vi "PicoScope5000aExampleStreamingMSO.vi"() -> ()   [LabVIEW 2010]
doc: "This example demonstrates how to use the PicoScope Labview library to stream data from a PicoScope 5000 Series Device"
uses:
  <vilib>/Waveform/DWDTOps.llb/DWDT Analog to Digital.vi
  PicoScope5000aLib/PicoScope5000aAnalogChannelSettings.ctl
  PicoScope5000aLib/PicoScope5000aDigitalChannelSettings.ctl
panel:
  in  "Port 0 Settings":T1={"Enabled"=FALSE, "Logic Level"=9830} {"Logic Level" items=["1.5V TTL"=9830, "2.5V CMOS"=16383]}
  in  "Channel A Settings":T2={"Enabled"=TRUE, "Coupling"=1, "Range"=6, "Analogue Offset"=0.0, "Bandwidth Limit"=0} {"Bandwidth Limit" items=["Full", "20MHz"]; "Range" items=["10 mV", "20 mV", "50 mV", "100 mV", "200 mV", "500 mV", "1 V", "2 V", "5 V", "10 V", "20 V"]; "Coupling" items=["AC", "DC"]}
  in  "Write ChA to file":bool
  out "Analog Channels":T3(graph)={0, "DownSample Interval (sec)"=1.600000020814234e-08, "Data"=[]}
  out "Raw Sample Interval (sec)":dbl format="%#.5p"
  out "Max ADC value":i16=32512
  out "Chunk time (ms)":u32
  out "Elapsed time (sec)":dbl
  in  "Data file":path=path "PicoScope5000aExampleStreaming ChA Data"
  out "Queue depth":i32(graph)=3
  out "queue depth":i32
  in  "Buffer and Transfer Settings":T4={"startIndex"=0, "Samples"=1000000, "Down Sample Ratio"=1, "Down-Sample Mode"=0} {"Down-Sample Mode" items=["None"=0, "Aggregate"=1, "Decimate"=2, "Average"=4]; "Down Sample Ratio" step=1; "Samples" format="%_6p"}
  out "USB Powered":bool=TRUE
  out "USB 3.0 device on non-USB 3.0 Port":bool
  out "TriggeredAt (In Buffer)":u32 format="%#.6p"
  out "TriggeredAt (Total samples)":u32 format="%#.6p"
  in  "Acquisition Settings":T5={"Auto Stop"=TRUE, "Desired Sample Interval"=1, "Pre-trigger Samples"=0, "Post-trigger Samples"=1000000, "Down-Sample Ratio"=1, "Down-Sample Mode"=0, "Time Units"=3} {"Time Units" items=["Nanoseconds (ns)"=2, "Microseconds (us)"=3, "Milliseconds (ms)"=4, "Seconds (s)"=5]; "Down-Sample Mode" items=["None"=0, "Aggregate"=1, "Decimate"=2, "Average"=4]; "Post-trigger Samples" format="%#.6p"; "Pre-trigger Samples" format="%#_6p"}
  out "Port 0":digitalwaveform(graph)={"t0"=timestamp(0 s since 1904-01-01), "dt"=1.600000020814234e-08, "Y"={"transitions"=[], "data"=[]}}
  in  "Trigger Settings":T6={"Trigger Enabled"=FALSE, "Trigger Source"=enum."Channel A", "Trigger Threshold (volts)"=0.0, "Trigger Direction"=2, "Trigger Delay (samples)"=0, "Auto Trigger Time (ms)"=1000} {"Trigger Direction" items=["Rising"=2, "Falling"=3]}
  out "Triggered":bool
  out "DownSample Interval (sec)":dbl format="%#.5p"
  out "Total Samples":u32 format="%#_5p"
  out "Auto Stopped":bool
  in  "Serial Number":string
  in  "Open Using Serial Number":bool
  out "Number of Samples per Capture":u32 format="%#.6p"
  in  "Resolution":u32(ring) items=["8-bit", "12-bit", "14-bit", "15-bit (max. 2 ch.)", "16-bit (max. 1 ch.)"]
  in  "Apply  Settings":bool
  in  "stop":bool
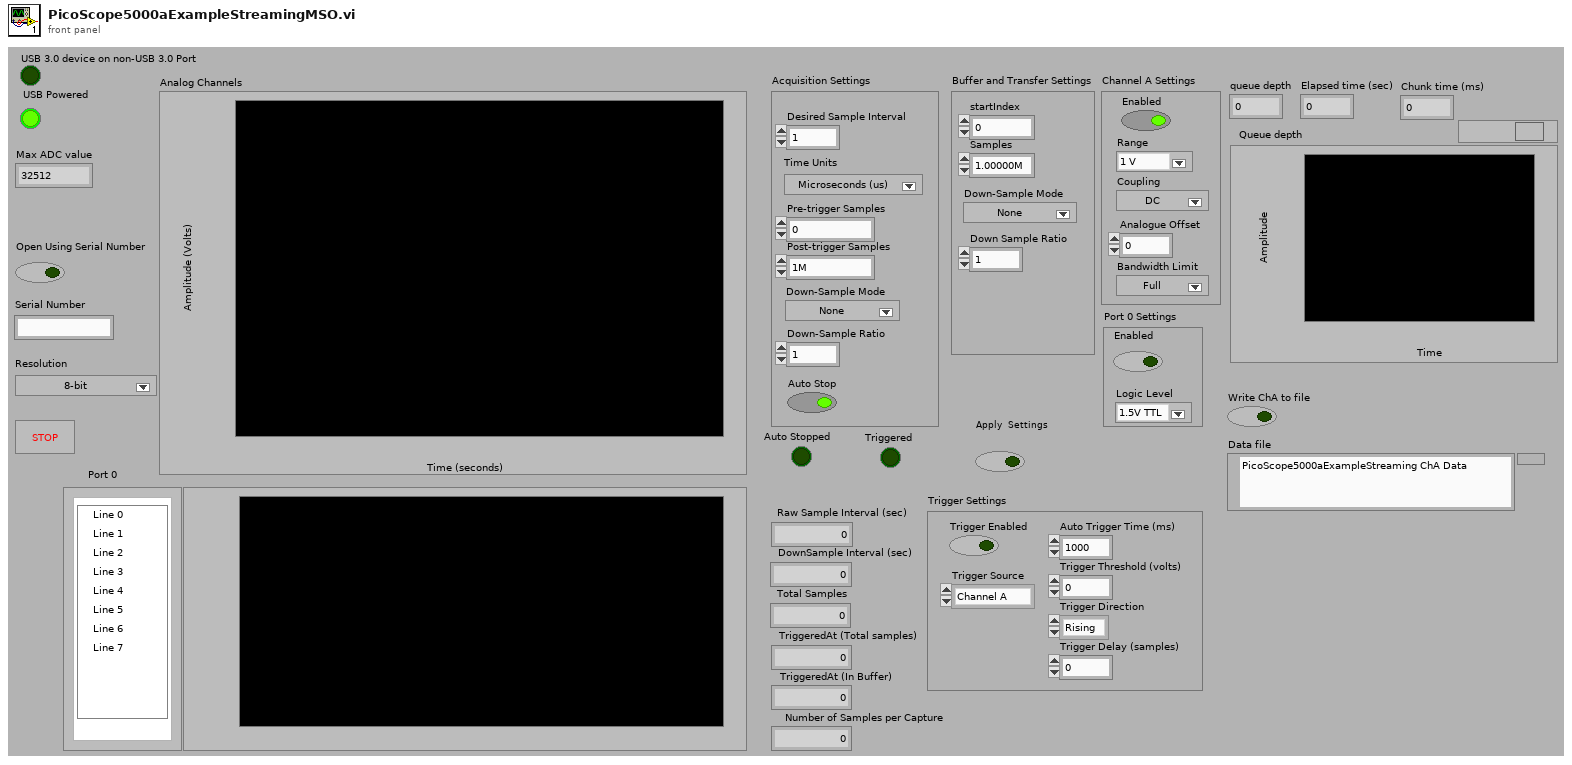
[diagram p1: front panel]
types:
  T1 = typedef "PicoScope5000aDigitalChannelSettings.ctl" = cluster{"Enabled":bool, "Logic Level":i16}
  T2 = typedef "PicoScope5000aAnalogChannelSettings.ctl" = cluster{"Enabled":bool, "Coupling":i16, "Range":u16, "Analogue Offset":sgl, "Bandwidth Limit":u32}
  T3 = cluster{i32, "DownSample Interval (sec)":dbl, "Data":dbl[]}
  T4 = cluster{"startIndex":u64, "Samples":u64, "Down Sample Ratio":u64, "Down-Sample Mode":u32}
  T5 = cluster{"Auto Stop":bool, "Desired Sample Interval":u32, "Pre-trigger Samples":u32, "Post-trigger Samples":u32, "Down-Sample Ratio":u32, "Down-Sample Mode":i32, "Time Units":u32}
  T6 = cluster{"Trigger Enabled":bool, "Trigger Source":enum16{"Channel A", "Channel B", "Channel C", "Channel D", "Ext."}, "Trigger Threshold (volts)":dbl, "Trigger Direction":u16, "Trigger Delay (samples)":u32, "Auto Trigger Time (ms)":i16}
  T7 = enum16{"open", "open or create", "create or replace", "create", "open (read-only)"}
  T8 = cluster{"Driver Version":string, "USB Version":string, "Hardware":string, "Variant":string, "Batch and Serial":string, "Cal Date":string, "Kernel Version":string, "Digital HW Version":string, "Analogue HW Version":string, "MSO":bool, "Number of channels":i16}
  T9 = cluster{"Channel A Buffer":i16[], "Channel B Buffer":i16[], "Channel C Buffer":i16[], "Channel D Buffer":i16[], "Channel E Buffer":i16[], "Channel F Buffer":i16[], "Channel G Buffer":i16[], "Channel H Buffer":i16[], "Port 0":i16[], "Port 1":i16[]}
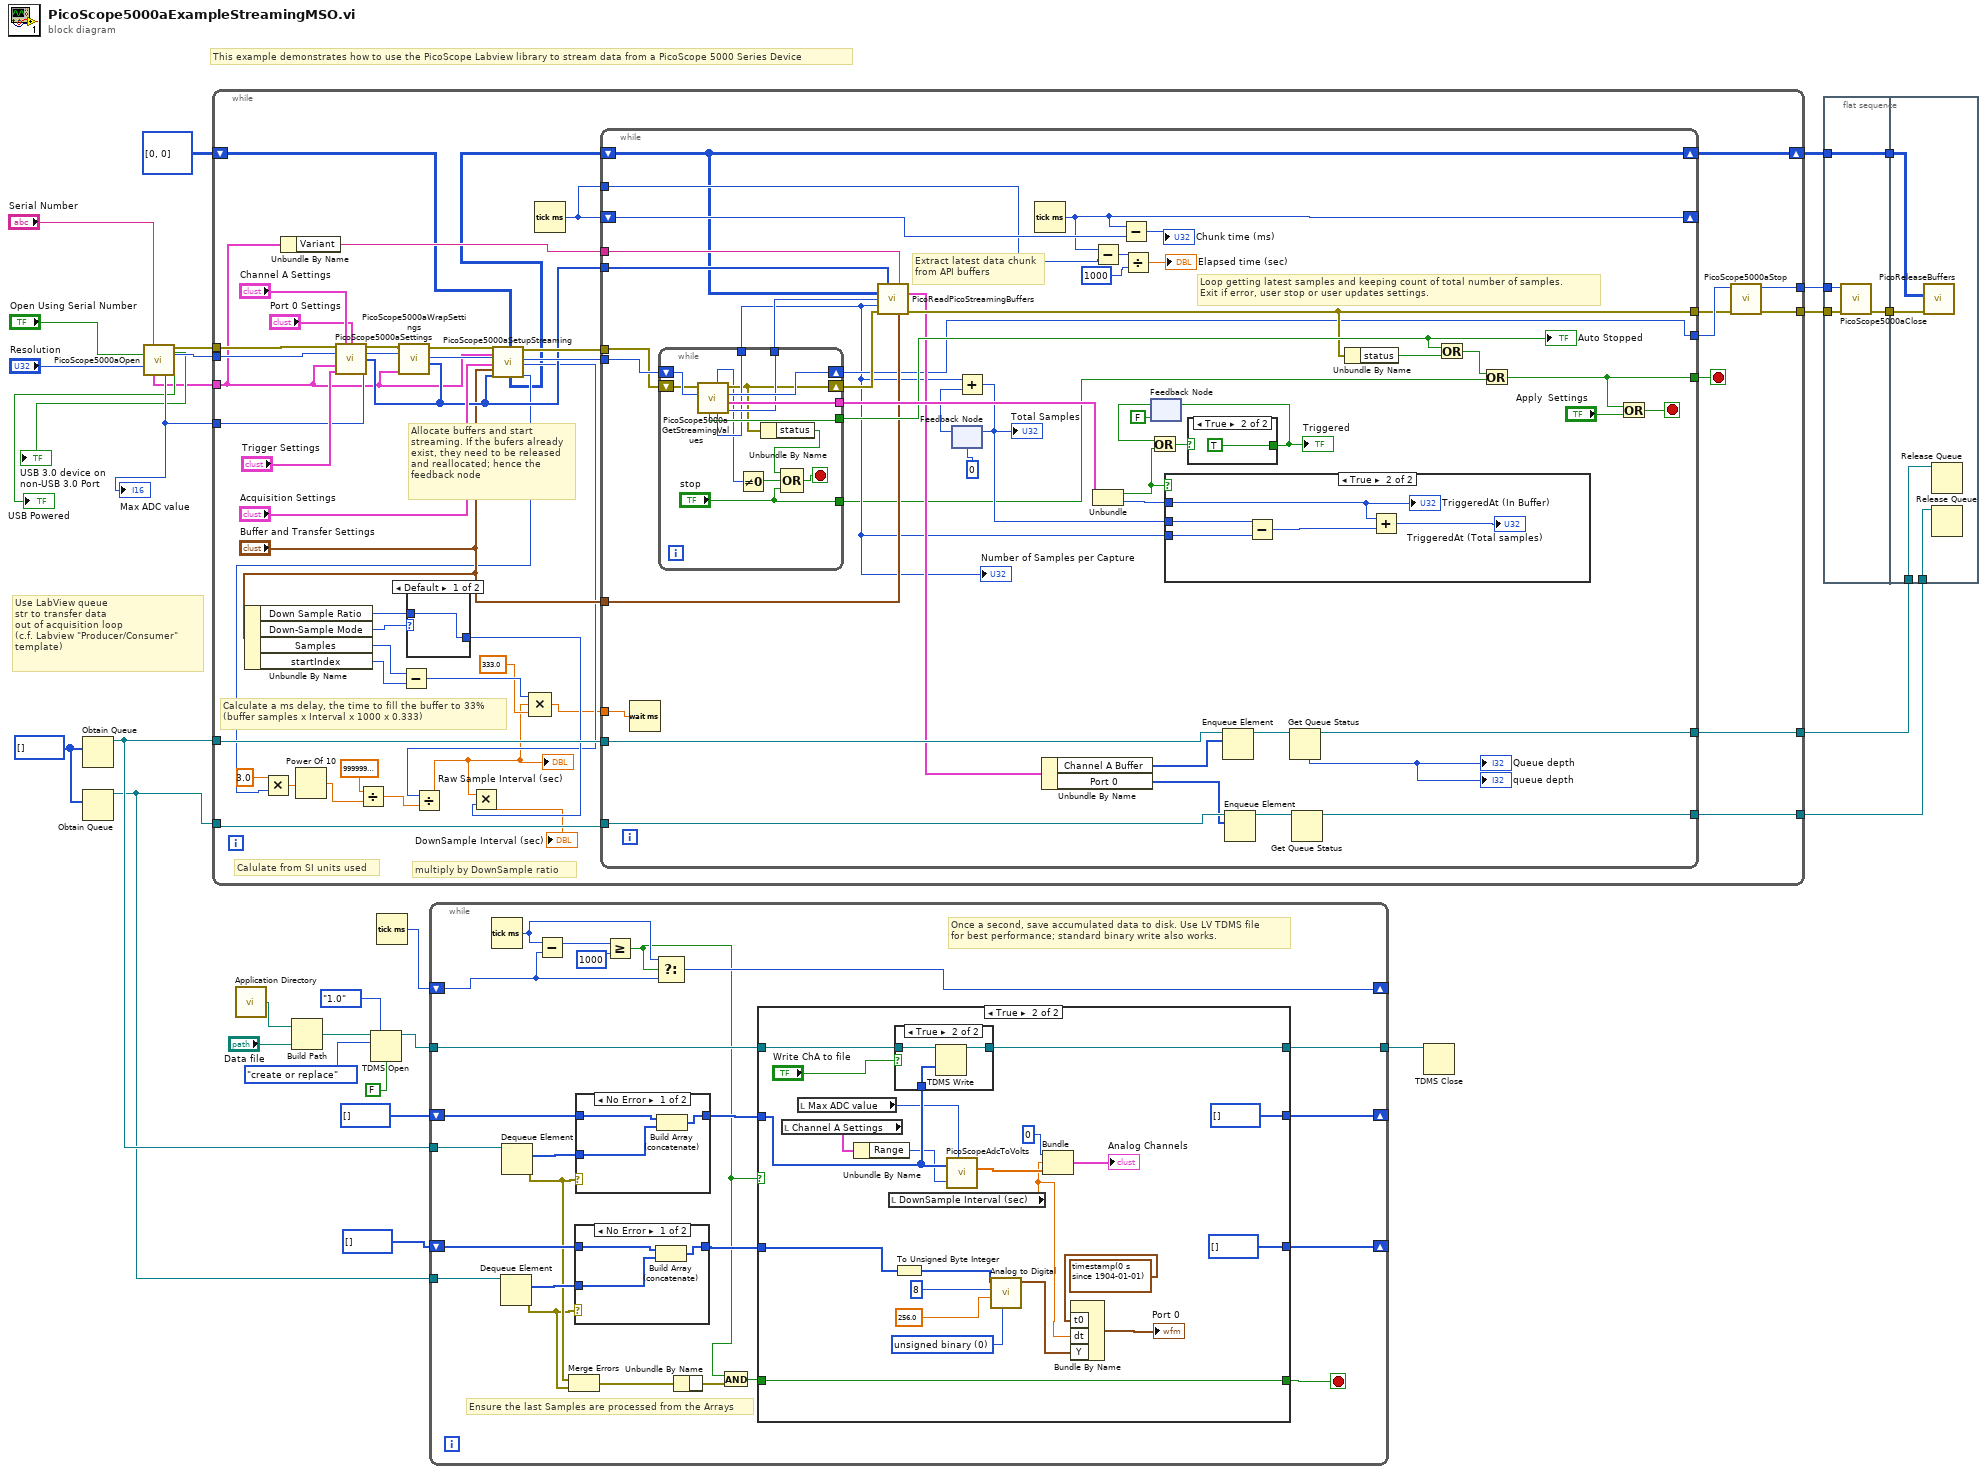
[diagram p0: block diagram]
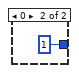
[diagram p6: hidden frame]
diagram:
  w15 = i16[] [] ("History Data")
  # "Use LabView queue\nstr to transfer data\nout of acquisition loop\n(c.f. Labview \"Producer/Consumer\"\ntemplate)"
  # "This example demonstrates how to use the PicoScope Labview library to stream data from a PicoScope 5000 Series Device"
  n1 = Obtain Queue(element data type=w15) -> (queue out=w25:refnum<queue>)  [unwired: 4 in, 2 out]
  n2 = Obtain Queue(element data type=w15) -> (queue out=w13:refnum<queue>)  [unwired: 4 in, 2 out]
  n3 = call "PicoScope5000aOpen.vi"("Serial Number"="Serial Number", "Use Serial Number"="Open Using Serial Number", "Resolution"="Resolution") -> ("USB 3.0 device on non-USB 3.0 Port"=→"USB 3.0 device on non-USB 3.0 Port":bool, "error out"=w31:errorcluster, "handle"=w30:i16, "USB Powered"=→"USB Powered":bool, "Device Info"=w8:T8, "Max ADC value"=w26:i16)  [unwired: 7 in]
  "Max ADC value" <- w26
  n4 = while {
    tunnel: w31 -> [w76]
    tunnel: w30 -> [w77]
    tunnel: w8 -> [w38]
    tunnel: w26 -> [w68]
    tunnel: [w62] -> w24
    tunnel: w25 -> [w61]
    tunnel: [w60] -> w14
    tunnel: w13 -> [w59]
    tunnel: [w36] -> w5
    tunnel: [w35] -> w4
    shift-right: [w34] -> w1
    shift-left: u64[][] [[0], [0]] ("Pointer array") -> [w33]
    stop <- w78 stop-if-true
    # "Calculate a ms delay, the time to fill the buffer to 33%\n(buffer samples x Interval x 1000 x 0.333)"
    # "Calulate from SI units used"
    # "multiply by DownSample ratio"
    # "Allocate buffers and start\nstreaming. If the bufers already\nexist, they need to be released\nand reallocated; hence the\nfeedback node"
    n5 = Unbundle By Name("Buffer and Transfer Settings") -> ("Down Sample Ratio"=w66:u64, "Down-Sample Mode"=w67:u32, "Samples"=w55:u64, "startIndex"=w54:u64)
    n6 = Unbundle By Name(w38) -> ("Variant"=w39:string)
    n7 = call "PicoScope5000aSettings.vi"("error in"=w76, "Channel A Settings"="Channel A Settings", "Port 0 Settings"="Port 0 Settings", "handle in"=w77, "Device Info"=w38, "Trigger Settings"="Trigger Settings", "Max ADC value"=w68) -> ("error out"=w71:errorcluster, "handle out"=w70:i16, "enabled array"=w64:i16[])  [unwired: 6 in]
    n8 = call "PicoScope5000aWrapSettings.vi"("enabled array"=w64, "Device Info"=w38, "Handle In"=w70, "error in (no error)"=w71) -> ("Handle Out"=w73:i16, "error out"=w72:errorcluster)  [unwired: 6 in]
    n9 = Subtract(x=w55, y=w54) -> (x-y=w44:u64)
    n10 = case shown="Default" w67 {
      tunnel: [w79 u32 1 ("Down-Sample Ratio")] -> w50
      tunnel: w66 -> [w79 _]
      frame Default {
      }
      frame 0 {
      }
    }
    n11 = call "PicoScope5000aSetupStreaming.vi"("error in"=w72, "Device Info"=w38, "handle in"=w73, "Acquisition Settings"="Acquisition Settings", "Buffer and Transfer Settings"="Buffer and Transfer Settings", "enabled array"=w64, "Pointers In"=w33) -> ("Pointer array"=w32:u64[][], "error out"=w74:errorcluster, "handle out"=w75:i16, "Sample Interval"=w46:u32, "sampleIntervalTimeUnits"=w48:u32)  [unwired: 8 in]
    n12 = Multiply(x=3.0, y=w48) -> (x*y=w53:dbl)
    n13 = Power Of 10(x=w53) -> (10^x=w52:dbl)
    n14 = Divide(x=sgl 1000000000000000.0 ("y"), y=w52) -> (x/y=w51:dbl)
    n15 = Divide(x=w46, y=w51) -> (x/y=w41:dbl)
    "Raw Sample Interval (sec)" <- w41
    n16 = Multiply(x=w41, y=w50) -> (x*y=→"DownSample Interval (sec)":dbl)
    n17 = Compound Arithmetic op=MULTIPLY(w44, w41, 333.0 ("value")) -> (w42:dbl)
    n18 = Tick Count (ms)() -> (millisecond timer value=w56:u32)
    n19 = while {
      tunnel: [w93] -> w58
      tunnel: [w125] -> w78
      tunnel: w75 -> [w110]
      tunnel: w74 -> [w109]
      tunnel: [w106] -> w57
      tunnel: "Buffer and Transfer Settings" -> [w108]
      tunnel: w64 -> [w105]
      tunnel: [w103] -> w62
      tunnel: w61 -> [w101]
      shift-right: [w95] -> _
      shift-left: w56 -> [w96]
      tunnel: w39 -> [w89]
      tunnel: [w87] -> w60
      tunnel: w59 -> [w86]
      tunnel: w56 -> [w83]
      tunnel: w42 -> [w82]
      shift-right: [w81] -> w34
      shift-left: w32 -> [w81]
      stop <- w124 stop-if-true
      # "Loop getting latest samples and keeping count of total number of samples. \nExit if error, user stop or user updates settings."
      # "Extract latest data chunk\nfrom API buffers"
      n20 = Wait (ms)(milliseconds to wait=w82) -> ()  [unwired: 1 out]
      n21 = while {
        tunnel: [w139] -> w123
        tunnel: [w138] -> w120
        tunnel: [w134] -> w91
        tunnel: [w133] -> w90
        shift-right: [w135] -> w93
        shift-left: w110 -> [w137]
        shift-right: [w132] -> w107
        shift-left: w109 -> [w136]
        tunnel: ["stop"] -> w84
        stop <- w128 stop-if-true
        n22 = call "PicoScope5000aGetStreamingValues.vi"("handle in"=w137, "error in"=w136) -> ("Start Index in Driver Buffer"=w134:u32, "Trigger"=w139:cluster{bool, "triggeredAt (Total samples)":u32}, "handle out"=w135:i16, "error out"=w132:errorcluster, "Number of Samples"=w133:u32, "ready"=w131:i16, "Auto Stopped"=w138:bool)  [unwired: 3 in]
        n23 = Not Equal To 0?(x=w131) -> (x != 0?=w129:bool)
        n24 = Unbundle By Name(w132) -> ("status"=w130:bool)
        n25 = Compound Arithmetic op=OR(w130, w129, "stop") -> (w128:bool)
      }
      "Number of Samples per Capture" <- w90
      "Auto Stopped" <- w120
      n26 = call "PicoReadPicoStreamingBuffers.vi"("enabled array"=w105, "Buffer and Transfer Settings"=w108, "Variant"=w89, "Pointer array"=w81, "Offset Index"=w91, "Number of Samples"=w90, "error in (no error)"=w107) -> ("Buffers (Max or non-aggregated)"=w100:T9, "error out"=w106:errorcluster)  [unwired: 6 in, 1 out]
      n27 = feedback #1(u32 0) -> (w116:u32)
      n28 = Add(x=w90, y=w116) -> (x+y=w114:u32)
      "Total Samples" <- w114
      n29 = feedback-in #1(w114) -> ()
      n30 = Tick Count (ms)() -> (millisecond timer value=w95:u32)
      n31 = Unbundle By Name(w100) -> ("Channel A Buffer"=w92:i16[], "Port 0"=w85:i16[])
      n32 = Subtract(x=w95, y=w83) -> (x-y=w99:u32)
      n33 = Unbundle(w123) -> (w112:bool, "triggeredAt (Total samples)"=w111:u32)
      n34 = Subtract(x=w95, y=w96) -> (x-y=→"Chunk time (ms)":u32)
      n35 = Divide(x=w99, y=u32 1000) -> (x/y=→"Elapsed time (sec)":dbl)
      n36 = feedback #2(FALSE) -> (w118:bool)
      n37 = Or(x=w118, y=w112) -> (x .or. y?=w115:bool)
      n38 = case shown="True" w112 {
        tunnel: w90 -> [_ w140]
        tunnel: w114 -> [_ w144]
        tunnel: w111 -> [_ w142]
        frame False {
        }
        frame True {
          n39 = Subtract(x=w144, y=w140) -> (x-y=w143:u32)
          n40 = Add(x=w142, y=w143) -> (x+y=→"TriggeredAt (Total samples)":u32)
          "TriggeredAt (In Buffer)" <- w142
        }
      }
      n41 = case shown="True" w115 {
        selector: w115 -> [w145 _]
        tunnel: [w145 TRUE] -> w113
        frame False {
        }
        frame True {
        }
      }
      "Triggered" <- w113
      n42 = feedback-in #2(w113) -> ()
      n43 = Enqueue Element(queue=w101, element=w92) -> (queue out=w102:refnum<queue>)  [unwired: 2 in, 2 out]
      n44 = Enqueue Element(queue=w86, element=w85) -> (queue out=w88:refnum<queue>)  [unwired: 2 in, 2 out]
      n45 = Get Queue Status(queue=w102) -> (queue out=w103:refnum<queue>, # elements in queue=→"queue depth" →"Queue depth":i32)  [unwired: 2 in, 6 out]
      n46 = Get Queue Status(queue=w88) -> (queue out=w87:refnum<queue>)  [unwired: 2 in, 7 out]
      n47 = Unbundle By Name(w106) -> ("status"=w122:bool)
      n48 = Or(x=w120, y=w122) -> (x .or. y?=w121:bool)
      n49 = Or(x=w121, y=w84) -> (x .or. y?=w125:bool)
      n50 = Or(x=w125, y="Apply  Settings") -> (x .or. y?=w124:bool)
    }
    n51 = call "PicoScope5000aStop.vi"("error in (no error)"=w57, "handle in"=w58) -> ("error out"=w36:errorcluster, "handle out"=w35:i16)  [unwired: 8 in]
  }
  n52 = call <vilib>:"Application Directory.vi"() -> ("Application Directory"=w9:path)
  n53 = Build Path(base path=w9, name or relative path="Data file") -> (appended path=w10:path)
  n54 = TDMS Open(6:FALSE ("disable buffering? (T)"), 7:enum16{"1.0", "2.0"}."1.0" ("file format version (2.0)"), 10:T7."create or replace" ("operation (0:open)"), 11:w10) -> (3:w19:refnum<k34>)  [unwired: 2 in, 1 out]
  n55 = Tick Count (ms)() -> (millisecond timer value=w21:u32)
  n56 = while {
    tunnel: w25 -> [w169]
    shift-right: [w162] -> _
    shift-left: i16[] [] ("History Data") -> [w168]
    shift-right: [w163] -> _
    shift-left: w21 -> [w164]
    tunnel: w19 -> [w161]
    tunnel: [w160] -> w18
    tunnel: w13 -> [w158]
    shift-right: [w155] -> _
    shift-left: i16[] [] ("History Data") -> [w157]
    stop <- w153 stop-if-true
    # "Ensure the last Samples are processed from the Arrays"
    # "Once a second, save accumulated data to disk. Use LV TDMS file\nfor best performance; standard binary write also works."
    n57 = Tick Count (ms)() -> (millisecond timer value=w165:u32)
    n58 = Dequeue Element(queue=w158) -> (element=w159:i16[], error out=w148:errorcluster)  [unwired: 2 in, 2 out]
    n59 = Dequeue Element(queue=w169) -> (element=w170:i16[], error out=w154:errorcluster)  [unwired: 2 in, 2 out]
    n60 = Subtract(x=w165, y=w164) -> (x-y=w167:u32)
    n61 = Merge Errors(w154, w148) -> (w150:errorcluster)
    n62 = case shown="No Error" w148 {
      tunnel: w157 -> [w173 w174]
      tunnel: [w172 w174] -> w156
      tunnel: w159 -> [w171 _]
      frame No Error {
        n63 = Build Array (concatenate)(w173, w171) -> (w172:i16[])
      }
      frame Error {
      }
    }
    n64 = case shown="No Error" w154 {
      tunnel: w168 -> [w207 w208]
      tunnel: [w206 w208] -> w152
      tunnel: w170 -> [w205 _]
      frame No Error {
        n65 = Build Array (concatenate)(w207, w205) -> (w206:i16[])
      }
      frame Error {
      }
    }
    n66 = Greater Or Equal?(x=w167, y=u32 1000) -> (x >= y?=w149:bool)
    n67 = Select(t=w165, s=w149, f=w164) -> (s? t:f=w163:u32)
    n68 = And(x=w149) -> (y=w147:errorcluster, x .and. y?=w151:bool)
    n69 = Unbundle By Name(w150, w147) -> ()
    n70 = case shown="True" w149 {
      tunnel: w152 -> [w178 w197]
      tunnel: [w178 i16[] [] ("History Data")] -> w162
      tunnel: w161 -> [w177 w199]
      tunnel: [w177 w198] -> w160
      tunnel: w156 -> [w176 w184]
      tunnel: [w176 i16[] [] ("History Data")] -> w155
      tunnel: [w175 w181] -> w153
      tunnel: w151 -> [w175 w181]
      frame False {
      }
      frame True {
        w190 = u16 0 items=["unsigned binary", "offset binary", "2's complement"] ("data format (offset binary)")
        n71 = local read "Channel A Settings"() -> (w179:T2)
        n72 = local read "Max ADC value"() -> (w193:i16)
        n73 = Unbundle By Name(w179) -> ("Range"=w196:u16)
        n74 = local read "DownSample Interval (sec)"() -> (w185:dbl)
        n75 = To Unsigned Byte Integer(number=w184) -> (unsigned 8bit integer=w189:u8[])
        n76 = case shown="True" "Write ChA to file" {
          tunnel: w199 -> [w201 w204]
          tunnel: [w201 w203] -> w198
          tunnel: w197 -> [_ w202]
          frame False {
          }
          frame True {
            n77 = TDMS Write(0:w204, 9:w202) -> (4:w203:refnum<k34>)  [unwired: 4 in, 3 out]
          }
        }
        n78 = call "PicoScopeAdcToVolts.vi"("Max_adc"=w193, "Range Index"=w196, "Data"=w197) -> ("Data"=w194:dbl[])
        n79 = call-poly <vilib>:"Analog to Digital.vi"("data format (offset binary)"=w190, "full-scale range (pk-pk)"=256.0, "resolution (16 bit)"=8, "analog waveform"=w189) -> ("digital waveform"=w186:digitalwaveform)  [unwired: 4 in, 3 out]
        n80 = Bundle(0, "DownSample Interval (sec)"=w185, "Data"=w194) -> (→"Analog Channels":T3)  [unwired: 1 in]
        n81 = Bundle By Name("t0"=timestamp(0 s since 1904-01-01), "dt"=w185, "Y"=w186) -> (→"Port 0":digitalwaveform)  [unwired: 1 in]
      }
    }
  }
  n82 = TDMS Close(11:w18) -> ()  [unwired: 1 in, 2 out]
  n83 = flat-sequence {
    tunnel: [w210] -> w7
    tunnel: w5 -> [w212]
    tunnel: w4 -> [w211]
    tunnel: [w209] -> w2
    tunnel: w1 -> [w209]
    tunnel: w24 -> [w216]
    tunnel: w14 -> [w215]
    tunnel: w7 -> [w214]
    tunnel: w2 -> [w213]
    frame #0 {
      n84 = call "PicoScope5000aClose.vi"("error in (no error)"=w212, "handle in"=w211) -> ("error out"=w210:errorcluster)  [unwired: 8 in, 1 out]
    }
    frame #1 {
      n85 = call "PicoReleaseBuffers.vi"("error in (no error)"=w214, "Pointer array"=w213) -> ()  [unwired: 8 in, 2 out]
      n86 = Release Queue(queue=w216) -> ()  [unwired: 2 in, 3 out]
      n87 = Release Queue(queue=w215) -> ()  [unwired: 2 in, 3 out]
    }
  }
